vi "Refnum to Session - Session to Refnum.vi"   [LabVIEW 2026]
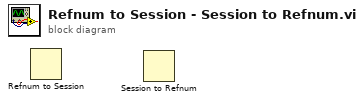
[diagram p0: block diagram]
diagram:
  n1 = Refnum to Session() -> ()  [unwired: 2 in, 2 out]
  n2 = Session to Refnum() -> ()  [unwired: 3 in, 2 out]
